vi "SemiGreedy_Filters_(Top_Level_VI)-6.vi"(5 "[IN] Max angle":dbl, 6 "[IN] Dot matrix with statuses \nfor potentially moving dots":i16[][](array[numeric]), 7 "[IN] Possibly\nMoving (X,Y)":dbl[][](array[numeric]), 8 "error IN":errorcluster, 9 "[IN] Areas particles\nPrimary Detected":dbl[][](array[numeric]), 10 "[IN] Primary \n(X,Y) Detected":dbl[][](array[numeric]), 11 "[IN] Grouped tracks":T1(array[cluster])) -> (0 "error OUT":errorcluster, 2 "[OUT] Processed Tracks":T1(array[cluster]), 3 "[OUT Tracks be\nfore Processing":T1(array[cluster]))   [LabVIEW 2017]
panel:
  out "Numeric":i32
  out "# Iteration":i32
  out "Current\ngroup":i32
  out "# of corrections":i32
  out "[IN] Before Pro\ncessing Tracks":T1(array[cluster])
  out "[IN] Current Pro\ncessing Tracks":T2
  out "[OUT] Clusters for Re\nconstructed Tracks":T2
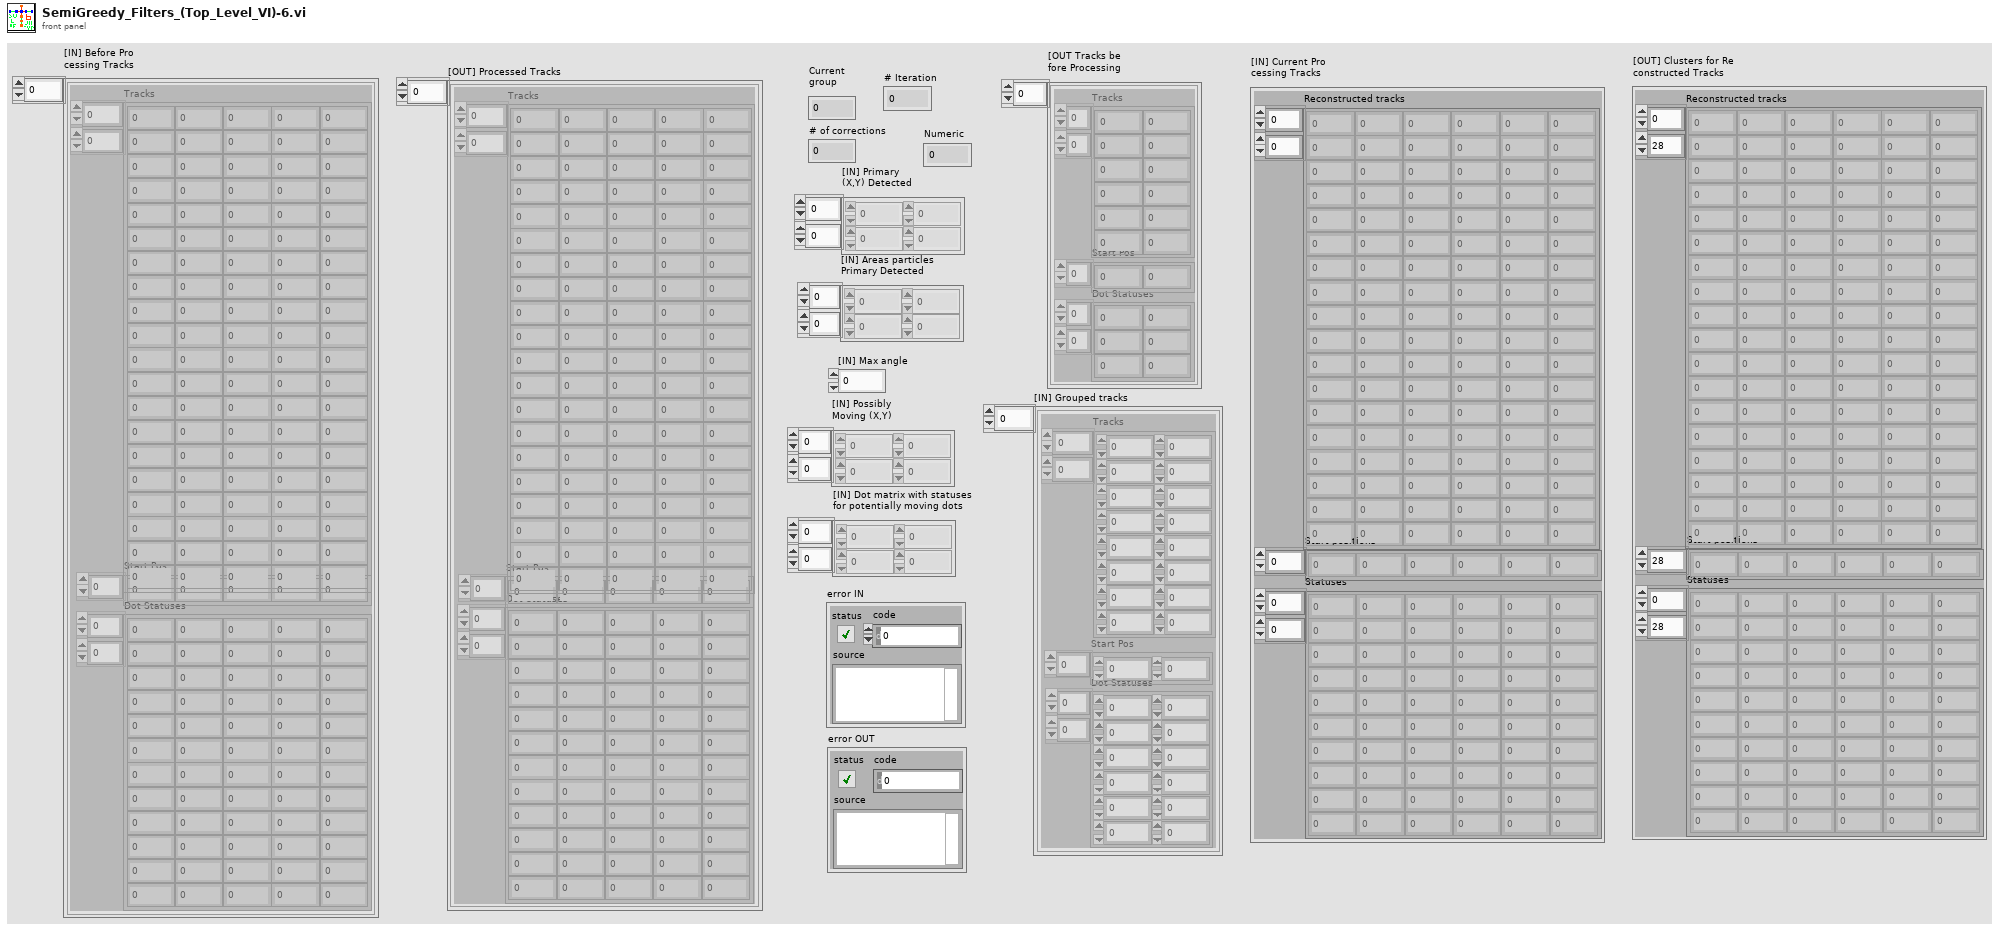
[diagram p1: front panel]
types:
  T1 = cluster{"Tracks":dbl[][], "Start Pos":i32[], "Dot Statuses":i16[][]}[]
  T2 = cluster{"Reconstructed tracks":dbl[][], "Start positions":i32[], "Statuses":i16[][]}
  T3 = cluster{"[IN] Possibly\nMoving (X,Y)":dbl[][], "[IN] Dot matrix with statuses \nfor potentially moving dots":i16[][], "[IN] Primary \n(X,Y) Detected ":dbl[][], "[IN] Max angle":dbl, "[IN] Areas particles\nPrimary Detected ":dbl[][]}
  T4 = cluster{"Tracks":dbl[][], "Start Pos":i32[], "Dot Statuses":i16[][]}
  T5 = cluster{"Subtrack":dbl[], "Statuses":i16[], "Start pos":i32, "Additions to cost":i8, "Track variant \nis too short":bool, "Indicies for Jumps":i32[]}[][]
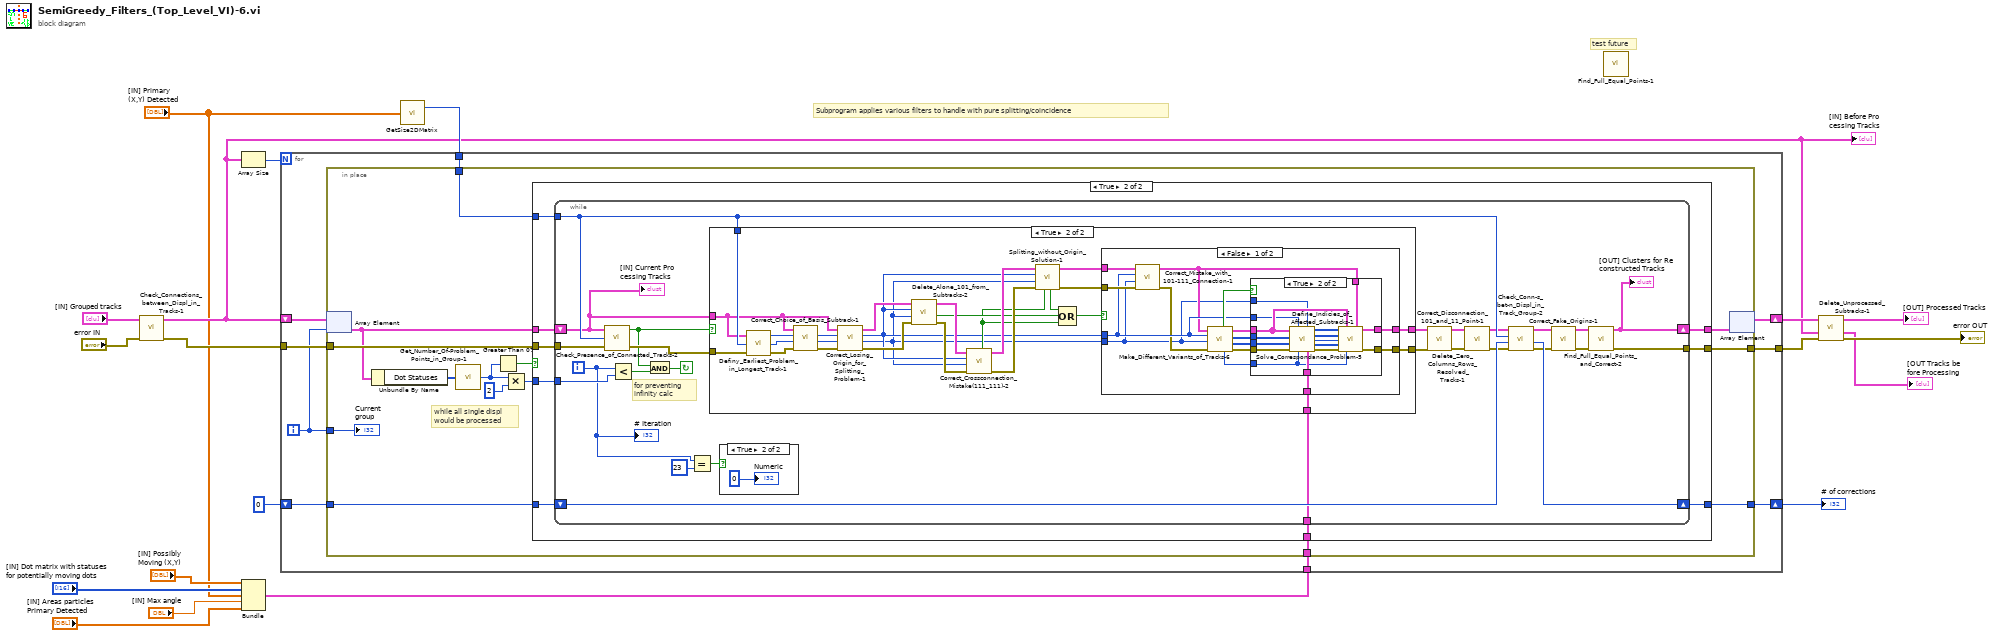
[diagram p0: block diagram]
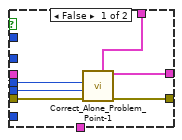
[diagram p5: hidden frame]
diagram:
  # "test future"
  # "Subprogram applies various filters to handle with pure splitting/coincidence"
  n1 = call "Check_Connections_between_Displ_in_Tracks-1.vi"("error IN"="error IN", "[IN] Long Connected Tracks"="[IN] Grouped tracks") -> ("error OUT"=w11:errorcluster, "[OUT] Long Connected Tracks"=w10:T1)  [unwired: 4 in]
  "[IN] Before Pro\ncessing Tracks" <- w10
  n2 = Array Size(array=w10) -> (size(s)=w19:i32)
  n3 = Bundle("[IN] Possibly\nMoving (X,Y)"="[IN] Possibly\nMoving (X,Y)", "[IN] Dot matrix with statuses \nfor potentially moving dots"="[IN] Dot matrix with statuses \nfor potentially moving dots", "[IN] Primary \n(X,Y) Detected"="[IN] Primary \n(X,Y) Detected", "[IN] Max angle"="[IN] Max angle", "[IN] Areas particles\nPrimary Detected"="[IN] Areas particles\nPrimary Detected") -> (w1:T3)  [unwired: 1 in]
  n4 = call "GetSize2DMatrix.vi"("Array IN (2D)"="[IN] Primary \n(X,Y) Detected") -> ("# Cols"=w16:i32)  [unwired: 1 out]
  n5 = for {
    N: w19 -> [_]
    shift-right: [w20] -> w15
    shift-left: w10 -> [w22]
    tunnel: w11 -> [w28]
    tunnel: w16 -> [w27]
    tunnel: [w26] -> w14
    shift-right: [w24] -> w7
    shift-left: 0 -> [w25]
    tunnel: w1 -> [w23]
    i -> [w21]
    n6 = in-place {
      in-place-border: w28 -> [w42]
      in-place-border: w27 -> [w41]
      in-place-border: [w40] -> w26
      in-place-border: w25 -> [w39]
      in-place-border: [w38] -> w24
      in-place-border: w23 -> [w35]
      in-place-border: w21 -> [w31]
      # "while all single displ\nwould be processed"
      n7 = in-place-array #1(w22, w21) -> (w30:T4)
      n8 = Unbundle By Name(w30) -> ("Dot Statuses"=w37:i16[][])
      n9 = call "Get_Number_Of-Problem_Points_in_Group-1.vi"("[IN] Dot Statuses"=w37) -> ("[OUT] Number of problem points"=w34:i32)
      n10 = Greater Than 0?(x=w34) -> (x > 0?=w36:bool)
      n11 = Multiply(x=w34, y=2) -> (x*y=w32:i32)
      n12 = case shown="True" w36 {
        tunnel: w42 -> [w44 w54]
        tunnel: w41 -> [_ w53]
        tunnel: [w44 w52] -> w40
        tunnel: [w45 w51] -> w29
        tunnel: w39 -> [w43 w50]
        tunnel: [w43 w49] -> w38
        tunnel: w30 -> [w45 w48]
        tunnel: w32 -> [_ w47]
        tunnel: w35 -> [_ w46]
        frame False {
        }
        frame True {
          n13 = while {
            tunnel: w54 -> [w73]
            tunnel: w53 -> [w70]
            shift-right: [w67] -> w51
            shift-left: w48 -> [w66]
            tunnel: [w69] -> w52
            shift-right: [w77] -> w49
            shift-left: w50 -> [w78]
            tunnel: w47 -> [w75]
            tunnel: w46 -> [w68]
            i -> [w59]
            stop <- w76 continue-if-true
            # "for preventing \ninfinity calc"
            n14 = call "Check_Presence_of_Connected_Tracks-2.vi"("error IN"=w73, "[IN] #of Frames"=w70, "[IN] Still connected\ntracks in group"=w66) -> ("error OUT"=w72:errorcluster, "[OUT] At least two tracks\ninside track group"=w71:bool)  [unwired: 1 in]
            n15 = Less?(x=w59, y=w75) -> (x < y?=w74:bool)
            n16 = And(x=w71, y=w74) -> (x .and. y?=w76:bool)
            n17 = Equal?(x=w59, y=23) -> (x = y?=w60:bool)
            n18 = case shown="True" w71 {
              tunnel: w72 -> [w82 w109]
              tunnel: w66 -> [w83 w88]
              tunnel: w70 -> [_ w108]
              tunnel: [w83 w107] -> w79
              tunnel: [w82 w106] -> w80
              tunnel: w68 -> [_ w102]
              frame False {
              }
              frame True {
                n19 = call "Definy_Earliest_Problem_in_Longest_Track-1.vi"("error IN"=w109, "[IN] #of Frames"=w108, "[IN] Still connected\ntracks in group"=w88) -> ("error OUT"=w103:errorcluster, "[OUT] # of Longest track\nInside the Group of Tracks"=w104:i32, "[OUT] Index of Problem\nPoint Inside Track"=w105:i32)
                n20 = call "Correct_Choice_of_Basis_Subtrack-1.vi"("error IN"=w103, "[IN] # of Longest track\nInside the Group of Tracks"=w104, "[IN] Index of Earliest \nProblem Point Inside"=w105, "[IN] Still connected\ntracks in group"=w88) -> ("error OUT"=w89:errorcluster, "[OUT] # of Correc\nted Longest Track"=w90:i32, "[OUT] # of Prob\nlem Point Inside"=w91:i32)  [unwired: 1 in]
                n21 = call "Correct_Losing_Origin_for_Splitting_Problem-1.vi"("error IN"=w89, "[IN] # of Correc\nted Longest Track"=w90, "[IN] # of Prob\nlem Point Inside"=w91, "[IN] Still connected\ntracks in group"=w88) -> ("error OUT"=w86:errorcluster, "[OUT] # of Correc\nted Longest Track"=w84:i32, "[OUT] # of Prob\nlem Point Inside"=w85:i32, "[OUT] Clusters for Re\nconstructed Tracks"=w87:T2)
                n22 = call "Delete_Alone_101_from_Subtracks-2.vi"("error IN"=w86, "[IN] # of Correc\nted Longest Track"=w84, "[IN] # of Prob\nlem Point Inside"=w85, "[IN] Still connected\ntracks in group"=w87) -> ("error OUT"=w98:errorcluster, "[OUT] Special case: \nAlone 101 point"=w93:bool, "[OUT] Clusters for Re\nconstructed Tracks"=w99:T2)  [unwired: 1 in]
                n23 = call "Correct_Crossconnection_Mistake(111_111)-2.vi"("error IN"=w98, "[IN] # of Track with\nFirst Problem Point"=w84, "[IN] Index of First Pro\nblem Point Inside Track"=w85, "[IN] Still connected\ntracks in group"=w99) -> ("error OUT"=w97:errorcluster, "[OUT] Clusters for Re\nconstructed Tracks"=w96:T2, "[OUT] Crossconn\nection corrected"=w92:bool)  [unwired: 5 in]
                n24 = call "Splitting_without_Origin_Solution-1.vi"("[IN] Crossconn\nection corrected"=w92, "error IN"=w97, "[IN] # of Track with\nFirst Problem Point"=w84, "[IN] Index of First Pro\nblem Point Inside Track"=w85, "[IN] Still connected\ntracks in group"=w96) -> ("error OUT"=w100:errorcluster, "[OUT] Clusters for Re\nconstructed Tracks"=w101:T2, "[OUT] Problem with 11 Point\nwithout Origin Resolved"=w95:bool)  [unwired: 4 in]
                n25 = Compound Arithmetic op=OR(w95, w93, w92) -> (w94:bool)
                n26 = case shown="False" w94 {
                  tunnel: [w118 w148] -> w107
                  tunnel: [w117 w147] -> w106
                  tunnel: w85 -> [w113 _]
                  tunnel: w84 -> [w110 _]
                  tunnel: w100 -> [w114 w147]
                  tunnel: w101 -> [w115 w148]
                  tunnel: w102 -> [w124 _]
                  frame False {
                    n27 = call "Correct_Mistake_with_101-111_Connection-1.vi"("error IN"=w114, "[IN] # of Correc\nted Longest Track"=w110, "[IN] # of Prob\nlem Point Inside"=w113, "[IN] Still connected\ntracks in group"=w115) -> ("error OUT"=w111:errorcluster, "[OUT] Clusters for Re\nconstructed Tracks"=w112:T2)  [unwired: 2 in]
                    n28 = call "Make_Different_Variants_of_Tracks-6.vi"("error IN"=w111, "[IN] # of Longest track\nInside the Group of Tracks"=w110, "[IN] Index of Earliest \nProblem Point Inside"=w113, "[IN] Still connected\ntracks in group"=w112) -> ("error OUT"=w123:errorcluster, "[OUT] Index of # tracks \nwith problem points"=w122:i32[], "[OUT] Index of connected \npoints inside the track"=w119:i32[], "[OUT] Subtracks"=w120:T5, "[OUT] Status of 1st Problem Point"=w121:i16, "[OUT] 2 or more subtracks"=w116:bool)  [unwired: 2 in]
                    n29 = case shown="True" w116 {
                      tunnel: w124 -> [_ w146]
                      tunnel: w123 -> [w127 w145]
                      tunnel: w122 -> [_ w144]
                      tunnel: w121 -> [_ w142]
                      tunnel: w120 -> [_ w139]
                      tunnel: w112 -> [w130 w138]
                      tunnel: w119 -> [_ w137]
                      tunnel: w113 -> [w126 w136]
                      tunnel: w110 -> [w125 w135]
                      tunnel: [w129 w132] -> w118
                      tunnel: [w128 w131] -> w117
                      frame False {
                        n30 = call "Correct_Alone_Problem_Point-1.vi"("[IN] # of Prob\nlem Point Inside"=w126, "[IN] # of Longest track\nInside the Group of Tracks"=w125, "error IN"=w127, "[IN] Still connected\ntracks in group"=w130) -> ("[OUT] Clusters for Re\nconstructed Tracks"=w129:T2, "error OUT"=w128:errorcluster)  [unwired: 3 in]
                      }
                      frame True {
                        n31 = call "Define_Indicies_of_Affected_Subtracks-1.vi"("[IN] Subtracks"=w139, "[IN] # of Prob\nlem Point Inside"=w136, "[IN] # of Longest track\nInside the Group of Tracks"=w135, "[IN] Index of connected \npoints inside the track"=w137, "[IN] Index of # tracks \nwith problem points"=w144, "error IN"=w145, "[IN] Status of 1st Problem Point"=w142, "[IN] Values for Cost F() Calc"=w146) -> ("[OUT] Indicies of \nPoints Inside Trks"=w133:i32[], "[OUT] Indicies of \nall Affected Tracks\n(initial point =0)"=w134:i32[], "[OUT] Index of Optimal \nSubtrack Splitting Case"=w141:i32, "[OUT] Optimal solution \nfor Merging Case"=w140:i32[], "error OUT"=w143:errorcluster)  [unwired: 3 in]
                        n32 = call "Solve_Correspondance_Problem-5.vi"("[IN] Indicies of Po\nints Inside Trks"=w133, "[IN] Subtracks"=w139, "[IN] Still connected\ntracks in group"=w138, "[IN] Indicies of all \nAffected Tracks \n(initial point = 0)"=w134, "[IN] Index of Optimal \nSubtrack Splitting Case"=w141, "[IN] Optimal solution \nfor Merging Case"=w140, "error IN"=w143, "[IN] Status of 1st \nProblem Point"=w142) -> ("[OUT] Clusters for Re\nconstructed Tracks"=w132:T2, "error OUT"=w131:errorcluster)  [unwired: 6 in]
                      }
                    }
                  }
                  frame True {
                  }
                }
              }
            }
            n33 = case shown="True" w60 {
              frame False {
              }
              frame True {
                "Numeric" <- 0
              }
            }
            n34 = call "Delete_Zero_Columns_Rows_Resolved_Tracks-1.vi"("error IN"=w80, "[IN] Clusters for Re\nconstructed Tracks"=w79) -> ("error OUT"=w64:errorcluster, "[OUT] Clusters for Re\nconstructed Tracks"=w65:T2)  [unwired: 4 in]
            n35 = call "Correct_Disconnection_101_and_11_Point-1.vi"("error IN"=w64, "[IN] Still connected\ntracks in group"=w65) -> ("error OUT"=w62:errorcluster, "[OUT] Clusters for Re\nconstructed Tracks"=w63:T2)  [unwired: 4 in]
            n36 = call "Check_Conn-s_bet-n_Displ_in_Track_Group-2.vi"("error IN"=w62, "[IN] # of Unconne\ncted Problem points"=w78, "[IN] #of Frames"=w70, "[IN] Clusters for Re\nconstructed Tracks"=w63) -> ("error OUT"=w58:errorcluster, "[OUT] # of Unconne\ncted Problem points"=w77:i32, "[OUT] Clusters for Re\nconstructed Tracks"=w57:T2)  [unwired: 1 in]
            n37 = call "Correct_Fake_Origins-1.vi"("error IN"=w58, "[IN] Still connected\ntracks in group"=w57) -> ("error OUT"=w55:errorcluster, "[OUT] Clusters for Re\nconstructed Tracks"=w56:T2)  [unwired: 4 in]
            n38 = call "Find_Full_Equal_Points_and_Correct-2.vi"("error IN"=w55, "[IN] Clusters for Re\nconstructed Tracks"=w56) -> ("error OUT"=w69:errorcluster, "[OUT] Clusters for Re\nconstructed Tracks"=w67:T2)  [unwired: 4 in]
            "[OUT] Clusters for Re\nconstructed Tracks" <- w67
            "# Iteration" <- w59
            "[IN] Current Pro\ncessing Tracks" <- w66
          }
        }
      }
      n39 = in-place-array #1(w29) -> (w20:T1)  [unwired: 1 out]
      "Current\ngroup" <- w31
    }
  }
  "# of corrections" <- w7
  n40 = call "Find_Full_Equal_Points-1.vi"() -> ()  [unwired: 6 in, 2 out]
  n41 = call "Delete_Unprocessed_Subtracks-1.vi"("error IN"=w14, "[IN] Before Pro\ncessing Tracks"=w10, "[IN] Processed Tracks"=w15) -> ("error OUT"=→"error OUT":errorcluster, "[OUT] Before Pro\ncessing Tracks"=→"[OUT Tracks be\nfore Processing":T1, "[IN] Filtered Tracks"=→"[OUT] Processed Tracks":T1)  [unwired: 2 in]
